vi "Close Engine Reference.vi"(4 "error in (no error)":errorcluster, 7 "EasyUserManager in":refnum<class "EasyUserManager.lvclass">) -> (0 "error out":errorcluster, 3 "EasyUserManager out":refnum<class "EasyUserManager.lvclass">)   [LabVIEW 2024, in "EasyUserManager.lvclass"]
doc: "This VI Closes the Teststand Engine Reference of an <B>Easy User Manager</B> object. \n\nCall this VI before stopping the main VI in LabVIEW or during clean-up in Teststand."
uses:
  EasyUserManager.lvclass
  EasyUserManager.lvclass/EasyUserManager.ctl
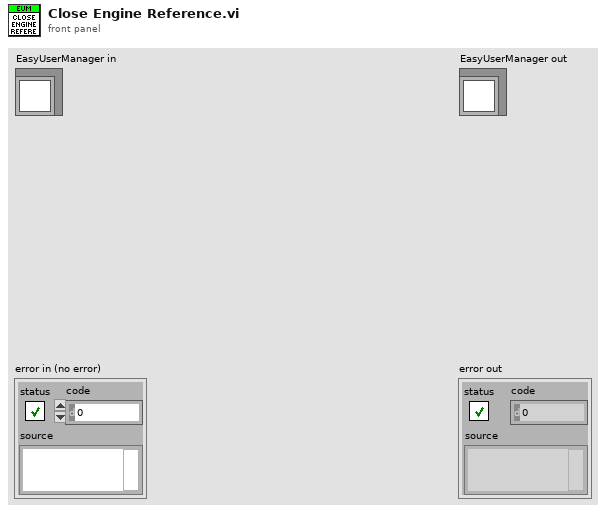
[diagram p1: front panel]
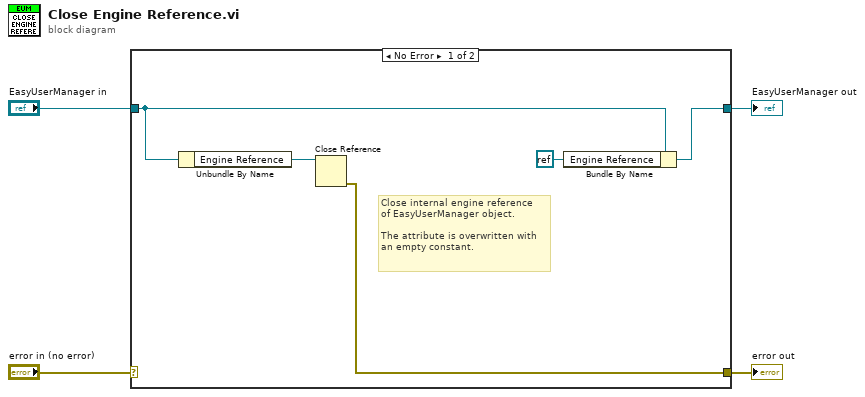
[diagram p0: block diagram]
diagram:
  n1 = case shown="No Error" "error in (no error)" {
    selector: "error in (no error)" -> [_ w11]
    tunnel: [w8 w11] -> w3
    tunnel: [w7 w10] -> w1
    tunnel: "EasyUserManager in" -> [w6 w10]
    frame No Error {
      # "Close internal engine reference\nof EasyUserManager object.\n\nThe attribute is overwritten with\nan empty constant."
      n2 = Unbundle By Name(w6) -> ("Engine Reference"=w9:refnum<k7>)
      n3 = Close Reference(reference=w9) -> (error out=w8:errorcluster)  [unwired: 1 in]
      n4 = Bundle By Name(cluster=w6, "Engine Reference"=refnum<k0> refnum) -> (w7:refnum<class "EasyUserManager.lvclass">)
    }
    frame Error {
      # "Pass error and do nothing."
    }
  }
  "error out" <- w3
  "EasyUserManager out" <- w1
